vi "Structured_Game_Data.vi"() -> (0 "Game Data":T1={"Close  Switch"=enum."Right", "Scale"=enum."Right", "Far Switch"=enum."Right"})   [LabVIEW 2017]
uses:
  TypeDef/Game_Data.ctl
  TypeDef/Plate_Positions.ctl
  TypeDef/Plate_Type.ctl
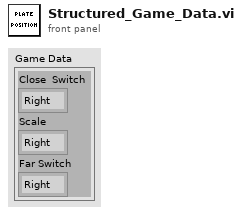
[diagram p1: front panel]
types:
  T1 = typedef "Game_Data.ctl" = cluster{"Close  Switch":T2, "Scale":T2, "Far Switch":T2}
  T2 = typedef "Plate_Positions.ctl" = enum16{"Left", "Right", "Unknown"}
  T3 = typedef "Plate_Type.ctl" = enum16{"Close Switch", "Scale", "Far Switch"}
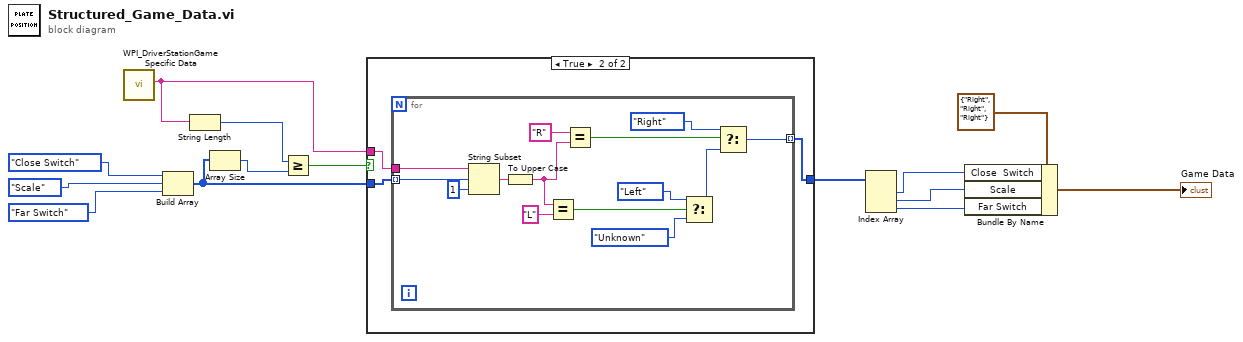
[diagram p0: block diagram]
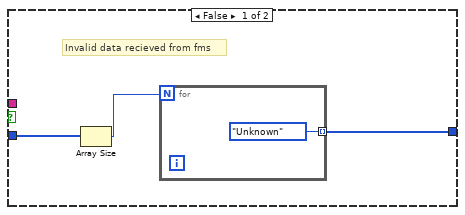
[diagram p2: hidden frame]
diagram:
  n1 = call <vilib>:"WPI_DriverStationGame Specific Data.vi"() -> ("Game Specific Data"=w4:string)  [unwired: 11 in]
  n2 = Build Array(Plate_Type."Close Switch" ("Plate Type"), Plate_Type."Scale" ("Plate Type"), Plate_Type."Far Switch" ("Plate Type")) -> (w5:T3[])
  n3 = String Length(string=w4) -> (length=w1:i32)
  n4 = Array Size(array=w5) -> (size(s)=w2:i32)
  n5 = Greater Or Equal?(x=w1, y=w2) -> (x >= y?=w3:bool)
  n6 = case shown="True" w3 {
    tunnel: w5 -> [w17 w21]
    tunnel: w4 -> [_ w20]
    tunnel: [w15 w19] -> w10
    frame False {
      # "Invalid data recieved from fms"
      n7 = Array Size(array=w17) -> (size(s)=w16:i32)
      n8 = for {
        N: w16 -> [_]
        tunnel: [Plate_Positions."Unknown" ("Plate Position")] -> w15 mode=indexing
      }
    }
    frame True {
      n9 = for {
        tunnel: w21 -> [w34] mode=indexing
        tunnel: w20 -> [w35]
        tunnel: [w22] -> w19 mode=indexing
        n10 = String Subset(string=w35, offset (0)=w34, length (rest)=1 ("length (rest)")) -> (substring=w32:string)
        n11 = To Upper Case(1:w32) -> (0:w30:string)
        n12 = Equal?(x=w30, y="L") -> (x = y?=w28:bool)
        n13 = Equal?(x="R", y=w30) -> (x = y?=w27:bool)
        n14 = Select(t=Plate_Positions."Left" ("Plate Position"), s=w28, f=Plate_Positions."Unknown" ("Plate Position")) -> (s? t:f=w26:T2)
        n15 = Select(t=Plate_Positions."Right", s=w27, f=w26) -> (s? t:f=w22:T2)
      }
    }
  }
  n16 = Index Array(array=w10) -> (element #1=w9:T2, element #2=w8:T2, element #3=w7:T2)  [unwired: 3 in]
  n17 = Bundle By Name(cluster=T1 {"Close  Switch"=enum."Right", "Scale"=enum."Right", "Far Switch"=enum."Right"}, "Close  Switch"=w9, "Scale"=w8, "Far Switch"=w7) -> (→"Game Data":T1)
